vi "Msg Action.vi"(0 "TCP Server in":refnum<class "TCP Server.lvclass">, 1 "TCP Client ID":refnum<k5>, 2 "Sender IP":string, 5 "TCP Server Msg Actions":T1, 7 "uService ID":string, 9 "uService Class Name":string, 11 "error in (no error)":errorcluster) -> (4 "TCP Server out":refnum<class "TCP Server.lvclass">, 6 "External Error out":errorcluster, 15 "error out":errorcluster)   [LabVIEW 2020, in "TALOS.lvlib" / "TCP Server.lvlib" / "TCP Server.lvclass"]
uses:
  TCP Server.lvclass
  TCP Server Msg Actions.ctl
  C:/LabVIEW Code/TALOS/builds/Actor Framework PPL/Actor Framework.lvlibp/1abvi3w/vi.lib/ActorFramework/Actor/Actor.lvclass
  C:/LabVIEW Code/TALOS/talos/Father of all uServices/Father of all uServices/Father of all uServices.lvclass
  Ancestor/Ancestor/Ancestor.lvclass/Ancestor.ctl
  Guardian/Guardian Messages/Launch uService Msg/Launch uService Msg.lvclass/Launch uService Msg.ctl
  Guardian/Guardian Messages/Message to uService Msg/Message to uService Msg.lvclass/Message to uService Msg.ctl
  Guardian/Guardian Messages/TCP-SV Message Interpreter Msg/TCP-SV Message Interpreter Msg.lvclass/TCP-SV Message Interpreter Msg.ctl
  Guardian/Guardian Messages/Message to uService Msg/Send Message to uService.vi
  FGV/Error Memory/Get Error Description.vi
  Ancestor/Ancestor/Read ID.vi
  Support VIs/Get Class Name.vi
  FGV/Error Memory/Error Memory Core.vi
  Support VIs/Circus Root Path.vi
  FGV/Error Memory/Error Crt Lvl checker.vi
  FGV/Error Memory/Error Memory Core.vi/40c8088d-b597-4017-91af-faa98e00292e.vi
  FGV/Error Memory/Error Memory Core.vi/d4a3ab98-063c-4e44-b43d-fbdcfe6c2be2.vi
  Father of all uServices/Father of all uServices/Father of all uServices.lvclass
  Support VIs/Global Memory.vi
  <vilib>/Utility/LVClass/Get LV Class Name.vi
  Support VIs/Is in Packed Library.vi
  Support VIs/TALOS Root path.vi
  Support VIs/Read CSV worksheet.vi
  Support VIs/Global Constants.vi
  <vilib>/Utility/error.llb/General Error Handler.vi
  <vilib>/Utility/config.llb/Open Config Data.vi
  <vilib>/Utility/config.llb/Get Section Names.vi
  <vilib>/Utility/config.llb/Get Key Names.vi
  <vilib>/Utility/config.llb/Read Key.vi
  <vilib>/Utility/config.llb/Read Key (String).vi
  <vilib>/Utility/config.llb/Close Config Data.vi
  builds/Actor Framework PPL/Actor Framework.lvlibp/1abvi3w/vi.lib/ActorFramework/Message Enqueuer/Enqueue.vi
  Support VIs/Error Log.vi
  Ancestor/Ancestor/Ancestor.lvclass
  <vilib>/Comparison/Equal/Equal Functor/Equal Functor.lvclass
  Guardian/Guardian Messages/Launch uService Msg/Launch uService Msg.lvclass
  Guardian/Guardian Messages/Message to uService Msg/Message to uService Msg.lvclass
  Guardian/Guardian Messages/TCP-SV Message Interpreter Msg/TCP-SV Message Interpreter Msg.lvclass
  builds/Actor Framework PPL/Actor Framework.lvlibp/1abvi3w/vi.lib/ActorFramework/Actor/Actor.lvclass
  TALOS.lvlib
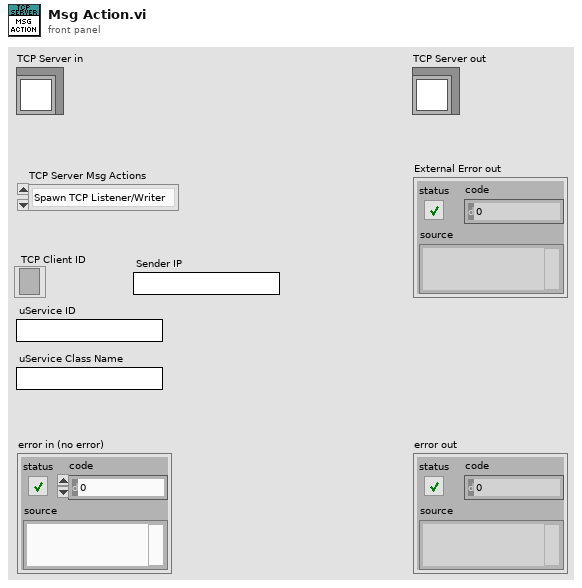
[diagram p1: front panel]
types:
  T1 = typedef "TALOS.lvlib/TCP Server.lvlib/TCP Server.lvclass/TCP Server Msg Actions.ctl" = enum16{"Spawn TCP Listener/Writer", "External Error", "I Exist", "Who the hell is this guy?", "Do nothing", "Are you the Bearer", "Farewell", "External Message"}
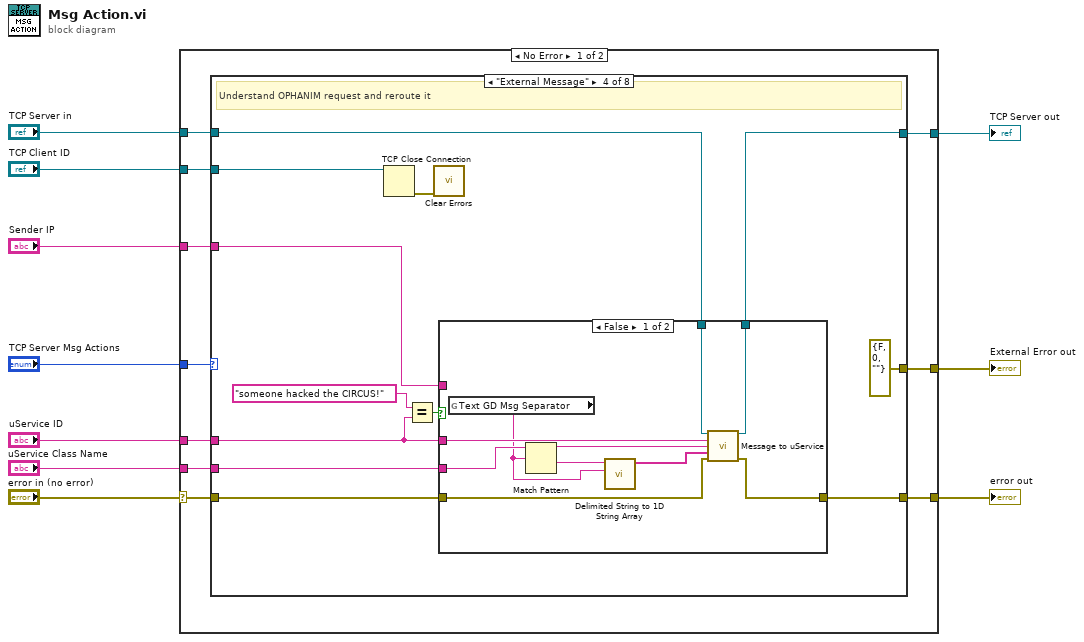
[diagram p0: block diagram]
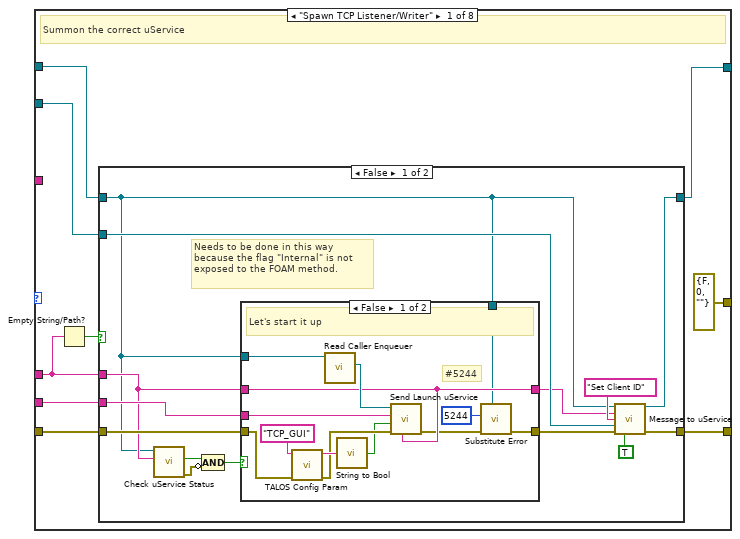
[diagram p2: hidden frame]
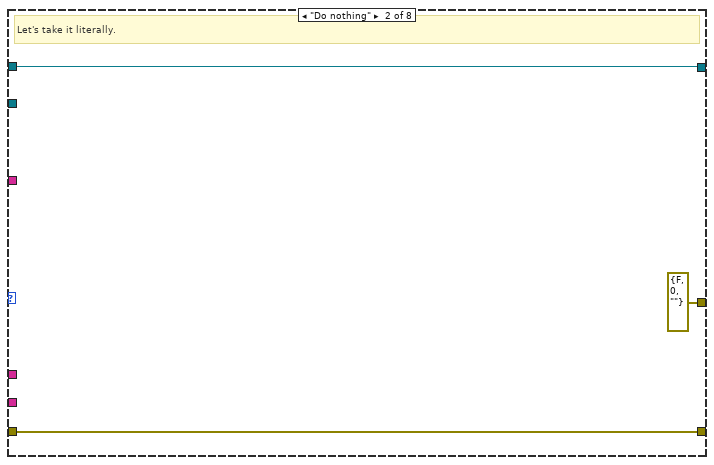
[diagram p5: hidden frame]
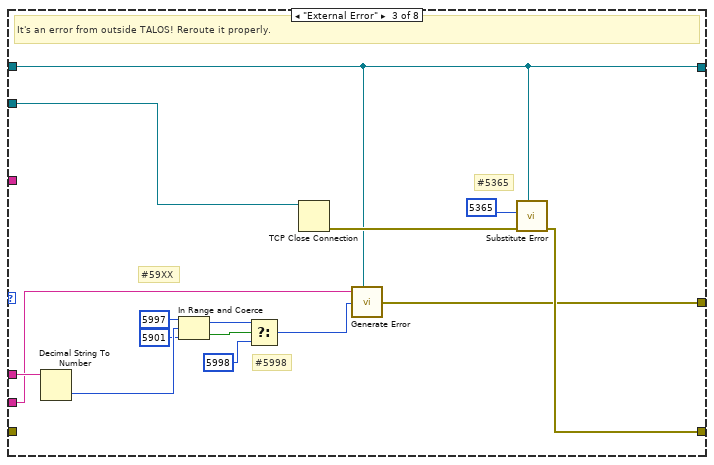
[diagram p6: hidden frame]
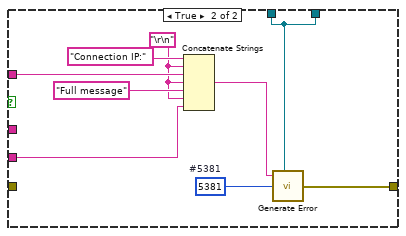
[diagram p7: hidden frame]
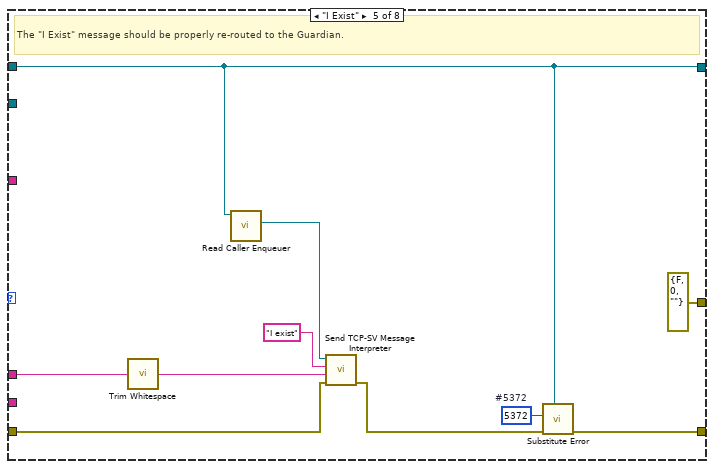
[diagram p8: hidden frame]
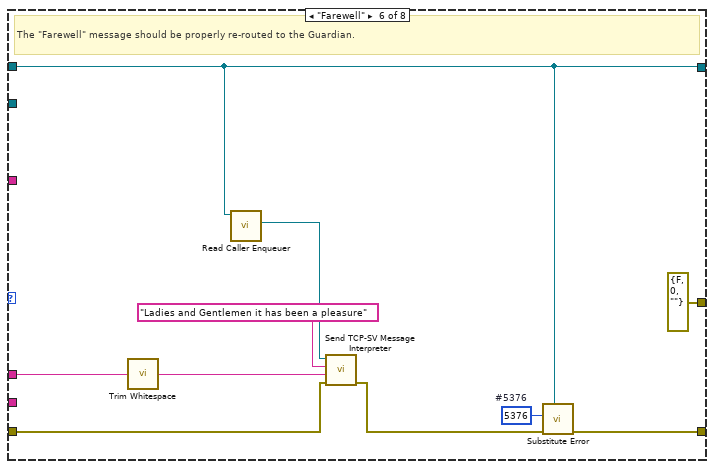
[diagram p9: hidden frame]
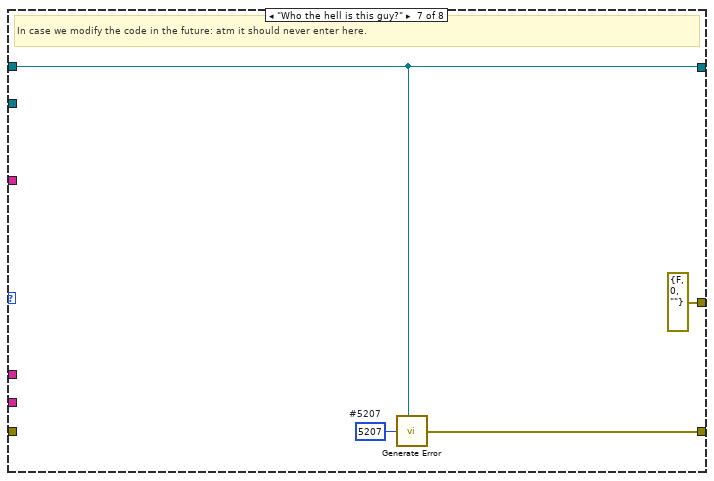
[diagram p10: hidden frame]
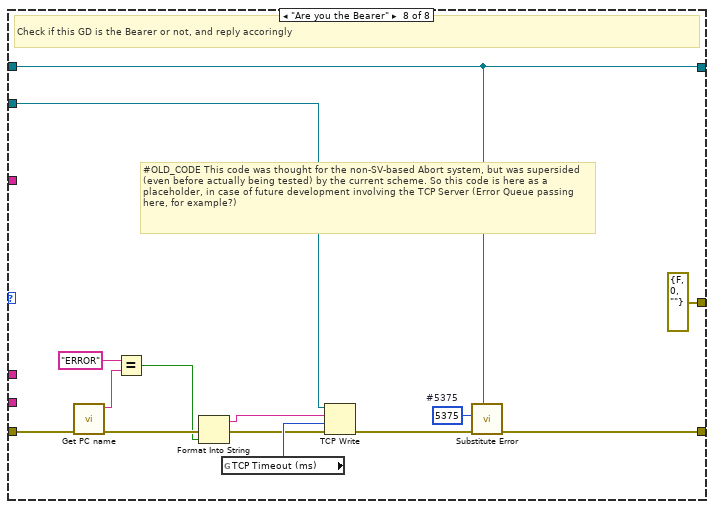
[diagram p11: hidden frame]
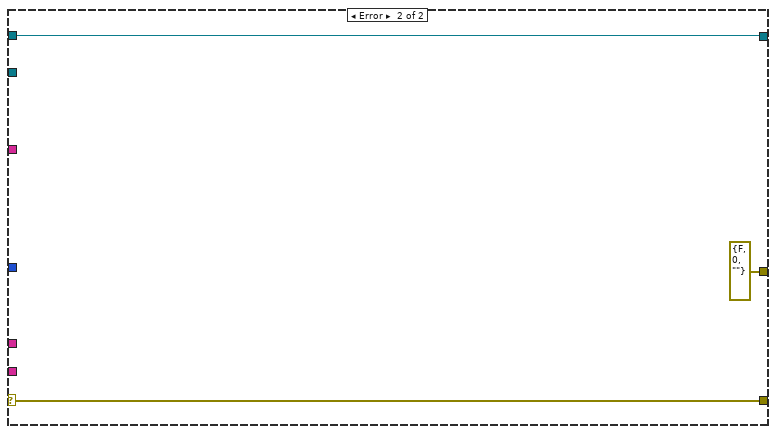
[diagram p12: hidden frame]
diagram:
  n1 = case shown="No Error" "error in (no error)" {
    selector: "error in (no error)" -> [w15 w149]
    tunnel: [w20 errorcluster {"status"=FALSE, "code"=0, "source"=""} ("error out")] -> w10
    tunnel: "TCP Server Msg Actions" -> [w19 _]
    tunnel: [w18 w150] -> w8
    tunnel: "uService Class Name" -> [w17 _]
    tunnel: "uService ID" -> [w16 _]
    tunnel: "TCP Server in" -> [w14 w150]
    tunnel: [w13 w149] -> w3
    tunnel: "TCP Client ID" -> [w12 _]
    tunnel: "Sender IP" -> [w11 _]
    frame No Error {
      n2 = case shown="\"External Message\"" w19 {
        tunnel: w12 -> [w29 _ w78 w90 _ _ _ w146]
        tunnel: [w28 w62 w74 w83 w114 w124 w132 w142] -> w13
        tunnel: w14 -> [w27 w63 w73 w86 w112 w122 w130 w141]
        tunnel: w15 -> [w26 w62 _ w84 w115 w125 _ w139]
        tunnel: w16 -> [w25 _ w77 w80 w117 w127 _ _]
        tunnel: w17 -> [w24 _ w76 w85 _ _ _ _]
        tunnel: [w22 w63 w73 w87 w112 w122 w130 w141] -> w18
        tunnel: [errorcluster {"status"=FALSE, "code"=0, "source"=""} ("error out") errorcluster {"status"=FALSE, "code"=0, "source"=""} ("error out") w64 errorcluster {"status"=FALSE, "code"=0, "source"=""} ("error out") errorcluster {"status"=FALSE, "code"=0, "source"=""} ("error out") errorcluster {"status"=FALSE, "code"=0, "source"=""} ("error out") errorcluster {"status"=FALSE, "code"=0, "source"=""} ("error out") errorcluster {"status"=FALSE, "code"=0, "source"=""} ("error out")] -> w20
        tunnel: w11 -> [_ _ _ w79 _ _ _ _]
        frame "Spawn TCP Listener/Writer" {
          # "Summon the correct uService"
          n3 = Empty String/Path?(string/path=w25) -> (empty?=w23:bool)
          n4 = case shown="False" w23 {
            tunnel: w27 -> [w30 w59]
            tunnel: w26 -> [w41 w60]
            tunnel: w24 -> [w40 _]
            tunnel: w25 -> [w31 _]
            tunnel: w29 -> [w38 _]
            tunnel: [w36 w60] -> w28
            tunnel: [w33 w59] -> w22
            frame False {
              # "Needs to be done in this way because the flag \"Internal\" is not exposed to the FOAM method."
              n5 = call-dynamic "Check uService Status.vi"("uService ID"=w31, "Father of all uServices in"=w30) -> ("error out"=w43:errorcluster, "Online?"=w32:bool)  [unwired: 6 in, 2 out]
              n6 = Compound Arithmetic op=AND(w32, invert w43) -> (w42:bool)
              n7 = case shown="False" w42 {
                tunnel: [w50 w58] -> w39
                tunnel: w30 -> [w56 _]
                tunnel: w41 -> [w46 w58]
                tunnel: w31 -> [w53 w57]
                tunnel: w40 -> [w54 _]
                tunnel: [w53 w57] -> w35
                tunnel: w30 -> [w49 _]
                frame False {
                  # "#5244"
                  # "Let's start it up"
                  n8 = call "TALOS Config Param.vi"("error in (no error)"=w46, "Parameter Name"="TCP_GUI") -> ("error out"=w45:errorcluster, "Output"=w48:string)  [unwired: 8 in]
                  n9 = call "Read Caller Enqueuer.vi"("Actor"=w56) -> ("Caller Enqueuer"=w55:refnum<class "Message Enqueuer.lvclass">)  [unwired: 10 in]
                  n10 = call "String to Bool.vi"("String"=w48) -> ("Boolean"=w44:bool)
                  n11 = call "Send Launch uService.vi"("uService ID"=w53, "error in (no error)"=w45, "GUI?"=w44, "uService Class Name"=w54, "Message Enqueuer"=w55) -> ("error out"=w51:errorcluster)  [unwired: 5 in, 1 out]
                  n12 = call "Substitute Error.vi"("LabVIEW Object"=w49, "error in (no error)"=w51, "Error Code"=5244) -> ("error out"=w50:errorcluster)  [unwired: 8 in]
                }
                frame True {
                  # "It's present!"
                }
              }
              n13 = call "Message to uService.vi"("Father of all uServices in"=w30, "uService ID"=w35, "Message"="Set Client ID" ("Item Name"), "Data"=w38, "error in (no error)"=w39, "Locale?"=TRUE) -> ("Father of all uServices out"=w33:refnum<class "TCP Server.lvclass">, "error out"=w36:errorcluster)  [unwired: 8 in]
            }
            frame True {
              # "We are in locale, or an error occurred, so do nothing!"
            }
          }
        }
        frame "Do nothing" {
          # "Let's take it literally."
        }
        frame "External Error" {
          # "#5998"
          # "#59XX"
          # "#5365"
          # "It's an error from outside TALOS! Reroute it properly."
          n14 = Decimal String To Number(string=w77) -> (number=w71:i32)  [unwired: 2 in, 1 out]
          n15 = In Range and Coerce(upper limit=5997, x=w71, lower limit=5901) -> (coerced(x)=w67:i32, In Range?=w68:bool)
          n16 = Select(t=w67, s=w68, f=5998) -> (s? t:f=w66:i32)
          n17 = TCP Close Connection(connection ID=w78) -> (error out=w75:errorcluster)  [unwired: 2 in, 1 out]
          n18 = call "Generate Error.vi"("Optional String"=w76, "Class"=w73, "Error Code"=w66) -> ("error out"=w64:errorcluster)  [unwired: 4 in]
          n19 = call "Substitute Error.vi"("LabVIEW Object"=w73, "error in (no error)"=w75, "Error Code"=5365) -> ("error out"=w74:errorcluster)  [unwired: 8 in]
        }
        frame "External Message" {
          # "Understand OPHANIM request and reroute it"
          n20 = TCP Close Connection(connection ID=w90) -> (error out=w88:errorcluster)  [unwired: 2 in, 1 out]
          n21 = Equal?(x="someone hacked the CIRCUS!", y=w80) -> (x = y?=w82:bool)
          n22 = call <vilib>:"Clear Errors.vi"("error in (no error)"=w88) -> ()  [unwired: 5 in, 2 out]
          n23 = case shown="False" w82 {
            tunnel: w80 -> [w100 _]
            tunnel: [w99 w109] -> w87
            tunnel: w86 -> [w98 w109]
            tunnel: w85 -> [w97 w102]
            tunnel: w84 -> [w95 _]
            tunnel: [w94 w108] -> w83
            tunnel: w79 -> [_ w105]
            frame False {
              n24 = global read "Global Constants.vi" "Text GD Msg Separator"() -> (w91:string)
              n25 = Match Pattern(string=w97, regular expression=w91) -> (before substring=w96:string, after substring=w92:string)  [unwired: 1 in, 2 out]
              n26 = call <vilib>:"Delimited String to 1D String Array.vi"("delimiter"=w91, "delimited string"=w92) -> ("string array"=w93:string[])  [unwired: 9 in]
              n27 = call "Message to uService.vi"("Father of all uServices in"=w98, "uService ID"=w100, "Message"=w96, "Data"=w93, "error in (no error)"=w95) -> ("Father of all uServices out"=w99:refnum<class "TCP Server.lvclass">, "error out"=w94:errorcluster)  [unwired: 9 in]
            }
            frame True {
              w103 = "\r\n"
              w107 = 5381  # #5381
              n28 = Concatenate Strings("Connection IP:" ("string"), w103, w105, w103, "Full message" ("string"), w103, w102) -> (w101:string)
              n29 = call "Generate Error.vi"("Optional String"=w101, "Class"=w109, "Error Code"=w107) -> ("error out"=w108:errorcluster)  [unwired: 4 in]
            }
          }
        }
        frame "I Exist" {
          w110 = 5372  # #5372
          # "The \"I Exist\" message should be properly re-routed to the Guardian."
          n30 = call <vilib>:"Trim Whitespace.vi"("string"=w117) -> ("trimmed string"=w116:string)  [unwired: 1 in]
          n31 = call "Read Caller Enqueuer.vi"("Actor"=w112) -> ("Caller Enqueuer"=w119:refnum<class "Message Enqueuer.lvclass">)  [unwired: 10 in]
          n32 = call "Send TCP-SV Message Interpreter.vi"("error in (no error)"=w115, "Data"=w116, "Message"="I exist", "Message Enqueuer"=w119) -> ("error out"=w113:errorcluster)  [unwired: 6 in, 1 out]
          n33 = call "Substitute Error.vi"("LabVIEW Object"=w112, "error in (no error)"=w113, "Error Code"=w110) -> ("error out"=w114:errorcluster)  [unwired: 8 in]
        }
        frame "Farewell" {
          w120 = 5376  # #5376
          # "The \"Farewell\" message should be properly re-routed to the Guardian."
          n34 = call <vilib>:"Trim Whitespace.vi"("string"=w127) -> ("trimmed string"=w126:string)  [unwired: 1 in]
          n35 = call "Read Caller Enqueuer.vi"("Actor"=w122) -> ("Caller Enqueuer"=w129:refnum<class "Message Enqueuer.lvclass">)  [unwired: 10 in]
          n36 = call "Send TCP-SV Message Interpreter.vi"("error in (no error)"=w125, "Data"=w126, "Message"="Ladies and Gentlemen it has been a pleasure", "Message Enqueuer"=w129) -> ("error out"=w123:errorcluster)  [unwired: 6 in, 1 out]
          n37 = call "Substitute Error.vi"("LabVIEW Object"=w122, "error in (no error)"=w123, "Error Code"=w120) -> ("error out"=w124:errorcluster)  [unwired: 8 in]
        }
        frame "Who the hell is this guy?" {
          w131 = 5207  # #5207
          # "In case we modify the code in the future: atm it should never enter here."
          n38 = call "Generate Error.vi"("Class"=w130, "Error Code"=w131) -> ("error out"=w132:errorcluster)  [unwired: 5 in]
        }
        frame "Are you the Bearer" {
          w144 = 5375  # #5375
          # "#OLD_CODE This code was thought for the non-SV-based Abort system, but was supersided (even before actually being tested) by the current scheme. So this code is here as a placeholder, in case of future development involving the TCP Server (Error Queue passing here, for example?)"
          # "Check if this GD is the Bearer or not, and reply accoringly"
          n39 = call "Get PC name.vi"("error in (no error)"=w139) -> ("error out"=w140:errorcluster, "Hostname"=w138:string)  [unwired: 9 in]
          n40 = Equal?(x="ERROR", y=w138) -> (x = y?=w136:bool)
          n41 = Format Into String(error in=w140, w136) -> (resulting string=w135:string, error out=w137:errorcluster)  [unwired: 2 in]
          n42 = global read "Global Constants.vi" "TCP Timeout (ms)"() -> (w147:i32)
          n43 = TCP Write(connection ID=w146, data in=w135, error in (no error)=w137, 9:w147) -> (error out=w143:errorcluster)  [unwired: 2 out]
          n44 = call "Substitute Error.vi"("LabVIEW Object"=w141, "error in (no error)"=w143, "Error Code"=w144) -> ("error out"=w142:errorcluster)  [unwired: 8 in]
        }
      }
    }
    frame Error {
    }
  }
  "External Error out" <- w10
  "TCP Server out" <- w8
  "error out" <- w3
